vi "test_lidar2.vi"() -> ()   [LabVIEW 2017]
panel:
  in  "Data":cluster{"Angle":dbl, dbl}[](array[cluster])
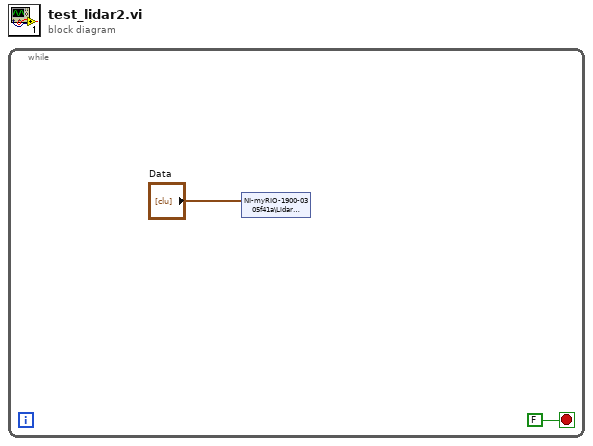
[diagram p0: block diagram]
diagram:
  n1 = while {
    stop <- FALSE stop-if-true
    n2 = shared-variable "NI-myRIO-1900-0305f41a\\Lidar Library.lvlib\\Data"("Data") -> ()  [unwired: 1 in, 1 out]
  }
